vi "OT Order Amplitude.vi"(5 "window ENBW (bins)":dbl=1.5, 6 "band half-width (orders)":dbl=0.2, 7 "order":dbl=1.0, 9 "delta order":dbl=0.1, 10 "order 0":dbl, 11 "magnitude":dbl[](array[numeric])) -> (3 "amplitude (EU rms)":dbl)   [LabVIEW 2026]
doc: "Amplitude of one order in a linear order power spectrum (same math as SVFA Power in Band).\namplitude (EU rms) = sqrt( sum of bins from order - half-width to order + half-width / window ENBW ).\nBins are rounded to the nearest index and clipped to the spectrum. Empty spectrum or a band outside it -> 0.\nwindow ENBW = 1.5 for Hanning (it undoes the window's spreading of one order over several bins)."
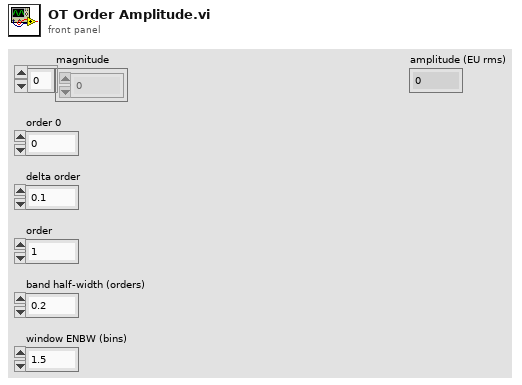
[diagram p1: front panel]
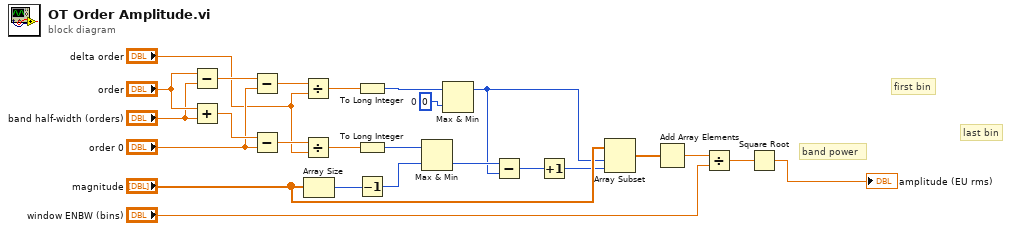
[diagram p0: block diagram]
diagram:
  w14 = 0  # 0
  # "band power"
  # "last bin"
  # "first bin"
  n1 = Subtract(x="order", y="band half-width (orders)") -> (x-y=w23:dbl)
  n2 = Add(x="order", y="band half-width (orders)") -> (x+y=w21:dbl)
  n3 = Subtract(x=w23, y="order 0") -> (x-y=w22:dbl)
  n4 = Subtract(x=w21, y="order 0") -> (x-y=w19:dbl)
  n5 = Divide(x=w22, y="delta order") -> (x/y=w17:dbl)
  n6 = Divide(x=w19, y="delta order") -> (x/y=w16:dbl)
  n7 = Array Size(array="magnitude") -> (size(s)=w13:i32)
  n8 = To Long Integer(number=w17) -> (32bit integer=w15:i32)
  n9 = To Long Integer(number=w16) -> (32bit integer=w12:i32)
  n10 = Decrement(x=w13) -> (x-1=w11:i32)
  n11 = Max & Min(x=w12, y=w11) -> (min(x,y)=w10:i32)  [unwired: 1 out]
  n12 = Max & Min(x=w15, y=w14) -> (max(x,y)=w7:i32)  [unwired: 1 out]
  n13 = Subtract(x=w10, y=w7) -> (x-y=w9:i32)
  n14 = Increment(x=w9) -> (x+1=w6:i32)
  n15 = Array Subset(array="magnitude", index=w7, length=w6) -> (w5:dbl[])
  n16 = Add Array Elements(numeric array=w5) -> (sum=w4:dbl)
  n17 = Divide(x=w4, y="window ENBW (bins)") -> (x/y=w2:dbl)
  n18 = Square Root(x=w2) -> (sqrt(x)=→"amplitude (EU rms)":dbl)
